vi "1_Waveform_Signal_Regression(Training).vi"() -> ()   [LabVIEW 2020]
uses:
  <vilib>/Ngene/Deep Learning Toolkit/Toolkit/NN_Train/Controls/NN_LR_Policy_Cfg.ctl
  <vilib>/Ngene/Deep Learning Toolkit/Toolkit/NN_Train/Controls/NN_LR_Policy_Type.ctl
  <vilib>/Ngene/Deep Learning Toolkit/Toolkit/NN_Train/Controls/NN_Train_Session_Data.ctl
  <vilib>/Ngene/Deep Learning Toolkit/Toolkit/NN_Train/Controls/NN_Train_Params.ctl
  <vilib>/Ngene/Deep Learning Toolkit/Toolkit/NN_Train/Controls/NN_Train_Optimizer.ctl
  <vilib>/Ngene/Deep Learning Toolkit/Toolkit/NN_Train/Controls/NN_Train_Data_Sampling.ctl
  <vilib>/Ngene/Deep Learning Toolkit/Toolkit/NN_Network/Controls/NN_Device.ctl
  <vilib>/Ngene/Deep Learning Toolkit/Toolkit/NN_Layers/Layers/Input/Controls/NN_Layer_Config(Input1D).ctl
  <vilib>/Ngene/Deep Learning Toolkit/Toolkit/NN_Data/Controls/NN_Data_type.ctl
  <vilib>/Ngene/Deep Learning Toolkit/Toolkit/NN_Layers/Layers/FC/Controls/NN_Layer_Config(FC).ctl
  <vilib>/Ngene/Deep Learning Toolkit/Toolkit/NN_Layers/Layers/BatchNorm/Controls/NN_BN_Params.ctl
  <vilib>/Ngene/Deep Learning Toolkit/Toolkit/NN_Activations/Controls/NN_Activation_Type.ctl
  <vilib>/Ngene/Deep Learning Toolkit/Toolkit/NN_Layers/Controls/NN_Layer_Init_Params.ctl
  <vilib>/Ngene/Deep Learning Toolkit/Toolkit/NN_Layers/Controls/NN_Layer_Weight_Init_Type.ctl
  <vilib>/Ngene/Deep Learning Toolkit/Toolkit/NN_Network/Controls/NN_Save_Before_Destroy_Options.ctl
  <vilib>/Ngene/Deep Learning Toolkit/Toolkit/NN_Layers/Layers/Input/NN_Layer_Create(Input1D).vi
  <vilib>/Ngene/Deep Learning Toolkit/Toolkit/NN_Layers/Layers/FC/NN_Layer_Create(FC).vi
  <vilib>/Ngene/Deep Learning Toolkit/Toolkit/NN_Train/Eval_Loss/NN_Eval_Test_Error_Loss/NN_Eval(In1D_Out1D).vi
  <vilib>/Ngene/Deep Learning Toolkit/Toolkit/NN_Train/Loss_Functions/NN_Set_Loss(MSE).vi
  <vilib>/Ngene/Deep Learning Toolkit/Toolkit/NN_Network/subVIs/NN_Predict/NN_Predict(In1D_Out1D).vi
  <vilib>/Ngene/Deep Learning Toolkit/Toolkit/Deep_Learning_Toolkit_by_Ngene.lvlib
  <vilib>/ptbypt/NI_PtbyPt.lvlib
panel:
  out "Training Loss":sgl=30.107077 format="%#.6g"
  in  "Eval":bool
  out "Loss Graphs":cluster{"mean":dbl, "Test Loss":sgl}(graph)
  in  "NN_Device":T1=enum."GPU"
  out "Test Loss":sgl=0.33381224 format="%#.6g"
  in  "Stop Training":bool
  in  "NN_Train_Params":T2={"Optimizer"=enum."Adam", "Beta_1"=0.9, "Beta_2"=0.999, "Weight Decay(L1)"=1e-07, "Weight Decay(L2)"=1e-07, "Data_Sampling"=enum."Random"}
  out "Session Data":T5={"Epochs"=22.1088, "Tot_Iter"=13818, "LR"=0.0025, "LR_iter"=13819}
  in  "LR Update Policy":T6={"Policy_Type"=enum."Step", "LR0"=0.010000000000000002, "k"=10.0, "WarmUp_Policy"=enum."Ramp", "WarmUp_Iter"=1000, "WarmUp_Ratio"=100.0} {"WarmUp_Ratio" min=1; "WarmUp_Iter" min=1; "LR0" format="%.7f"}
  # "Overview: This example demonstrating the usage of Deep Learning Toolkit for solving  waveform signal regression problem.\nRequirements: Deep Learning Toolkit for LabVIEW\nInstructions:\n1.  Run the VI with current configuration of the training parameters and Learning Rate update policy.\n2. Observe how the training loss is decreasing.\n3. Press the \"Stop Training\" when the loss is not decreasing any more."
  # "Waveform Signal Regression (Frequency Prediction) - Training"
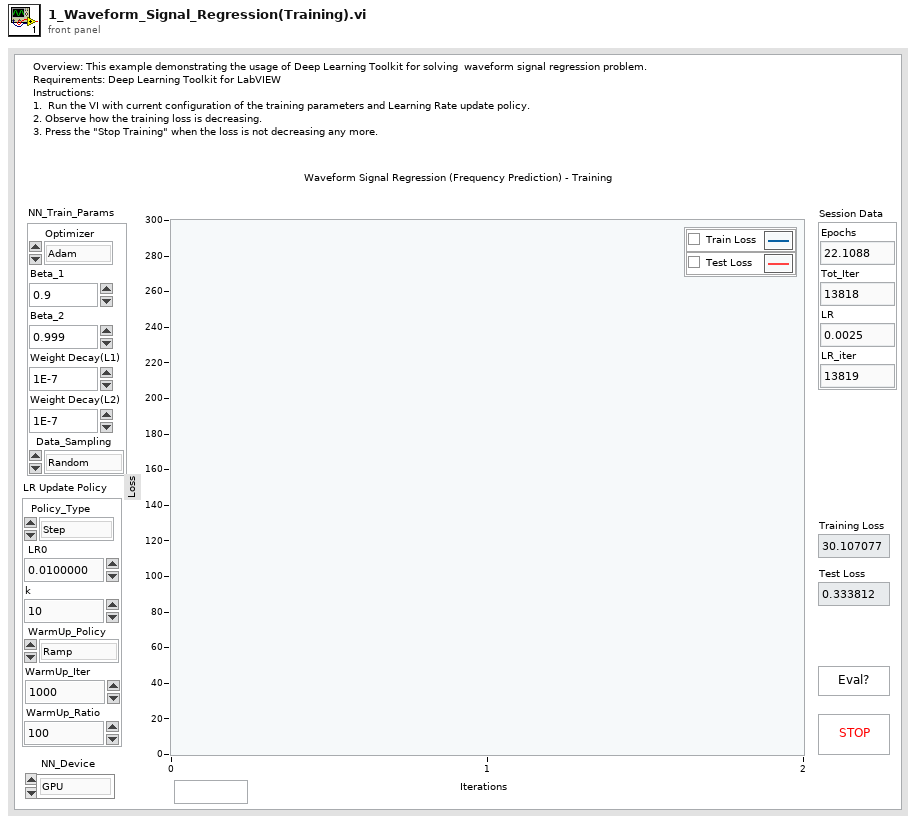
[diagram p1: front panel]
types:
  T1 = typedef "Deep_Learning_Toolkit_by_Ngene.lvlib/NN_Device.ctl" = enum16{"CPU", "GPU"}
  T2 = typedef "Deep_Learning_Toolkit_by_Ngene.lvlib/NN_Train_Params.ctl" = cluster{"Optimizer":T3, "Beta_1":sgl, "Beta_2":sgl, "Weight Decay(L1)":sgl, "Weight Decay(L2)":sgl, "Data_Sampling":T4}
  T3 = typedef "Deep_Learning_Toolkit_by_Ngene.lvlib/NN_Train_Optimizer.ctl" = enum16{"SGD", "Adam", "Adagrad", "Adadelta", "RMSProp", "Nesterov"}
  T4 = typedef "Deep_Learning_Toolkit_by_Ngene.lvlib/NN_Train_Data_Sampling.ctl" = enum16{"Random", "Sequential"}
  T5 = typedef "Deep_Learning_Toolkit_by_Ngene.lvlib/NN_Train_Session_Data.ctl" = cluster{"Epochs":sgl, "Tot_Iter":i32, "LR":sgl, "LR_iter":i32}
  T6 = typedef "Deep_Learning_Toolkit_by_Ngene.lvlib/NN_LR_Policy_Cfg.ctl" = cluster{"Policy_Type":T7, "LR0":dbl, "k":sgl, "WarmUp_Policy":enum16{"Step", "Ramp"}, "WarmUp_Iter":i32, "WarmUp_Ratio":sgl}
  T7 = typedef "Deep_Learning_Toolkit_by_Ngene.lvlib/NN_LR_Policy_Type.ctl" = enum16{"Manual", "Step", "Exp", "1/t"}
  T8 = typedef "Deep_Learning_Toolkit_by_Ngene.lvlib/NN_Save_Before_Destroy_Options.ctl" = cluster{"CFG?":bool, "Weights?":bool, "Render?":bool}
  T9 = typedef "Deep_Learning_Toolkit_by_Ngene.lvlib/NN_Layer_Config(FC).ctl" = cluster{"Name":string, "Size":i32, "BN":bool, "BN_Params":T10, "Activation":T11, "Has Bias?":bool, "Init_Params":T12, "Custom_Params":string}
  T10 = typedef "Deep_Learning_Toolkit_by_Ngene.lvlib/NN_BN_Params.ctl" = cluster{"epsilon":sgl, "momentum":sgl}
  T11 = typedef "Deep_Learning_Toolkit_by_Ngene.lvlib/NN_Activation_Type.ctl" = enum16{"Sigmoid", "ReLU", "LReLU", "ReLU6", "GELU", "tanh", "Swish", "Mish", "None"}
  T12 = typedef "Deep_Learning_Toolkit_by_Ngene.lvlib/NN_Layer_Init_Params.ctl" = cluster{"Init_Type":T13, "Value":sgl}
  T13 = typedef "Deep_Learning_Toolkit_by_Ngene.lvlib/NN_Layer_Weight_Init_Type.ctl" = enum16{"Const", "Uniform", "Gaussian", "Xavier"}
  T14 = typedef "Deep_Learning_Toolkit_by_Ngene.lvlib/NN_Layer_Config(Input1D).ctl" = cluster{"Name":string, "Size":i32, "Data_Type":T15, "Shift":sgl, "Scale":sgl}
  T15 = typedef "Deep_Learning_Toolkit_by_Ngene.lvlib/NN_Data_type.ctl" = enum16{"I8", "U8", "I16", "U16", "U32 ARGB", "SGL"}
  T16 = typedef "Deep_Learning_Toolkit_by_Ngene.lvlib/NN_DataSets_All(In1D_Out1D).ctl" = cluster{"Train":T17, "Validation":T17, "Test":T17}
  T17 = typedef "Deep_Learning_Toolkit_by_Ngene.lvlib/NN_DataSet(In1D_Out1D).ctl" = cluster{"Inputs Ref.":variant, "Outputs Ref.":T18, "Dims_In":i32, "Dataset_Size":i32, "Dims_Out":i32, "Labels":string[], "File Paths":path[], "Custom_Data":variant}
  T18 = typedef "Deep_Learning_Toolkit_by_Ngene.lvlib/NN_Data_ref(2D_SGL).ctl" = refnum<data-value>
  T19 = typedef "Deep_Learning_Toolkit_by_Ngene.lvlib/NN.ctl" = cluster{"Name":string, "No of Layers":i32, "mBatch":i32, "Layers":T20[], "Dimty":T21, "Dims_In":T22, "Dims_Out":T22, "Working_Dir":path, "Train?":bool, "Train_Params":T2, "LR_Update_Policy":T6, "Session Data":T5, "Ground_truth":T23, "NNg_hdls":T24, "NN_Device":T1, "GPU Id":i32, "Labels":string[], "Loss_Type":T25, "Loss_Cfg_Prms":variant, "NNG_WS":T26, "DryRun?":bool}
  T20 = typedef "Deep_Learning_Toolkit_by_Ngene.lvlib/NN_Layer_ref.ctl" = refnum<file>
  T21 = typedef "Deep_Learning_Toolkit_by_Ngene.lvlib/NN_In_Out_Dim-ty.ctl" = enum8{"In1D_Out1D", "In3D_Out1D", "In3D_Out3D", "In3D_OutBBox"}
  T22 = typedef "Deep_Learning_Toolkit_by_Ngene.lvlib/NN_Dims(C,H,W).ctl" = cluster{"C":i32, "H":i32, "W":i32}
  T23 = typedef "Deep_Learning_Toolkit_by_Ngene.lvlib/NN_Ground_truth.ctl" = cluster{"Y":variant}
  T24 = typedef "Deep_Learning_Toolkit_by_Ngene.lvlib/nng_cuda_handles.ctl" = cluster{"cudnn":u64, "cublas":u64, "stream":u64, "curand":u64}
  T25 = typedef "Deep_Learning_Toolkit_by_Ngene.lvlib/NN_Loss_Type.ctl" = enum16{"None", "MSE", "CrossEntropy", "YOLO_v2", "YOLO_v4"}
  T26 = typedef "Deep_Learning_Toolkit_by_Ngene.lvlib/NNG_WS.ctl" = cluster{"NNG_WS_Mem":T27, "Max_WS_Size":i64}
  T27 = typedef "Deep_Learning_Toolkit_by_Ngene.lvlib/NNg_WS_Mem_DVR.ctl" = refnum<data-value>
  T28 = typedef "Deep_Learning_Toolkit_by_Ngene.lvlib/NN_Eval_Params.ctl" = cluster{"Loss":sgl, "Error":sgl}
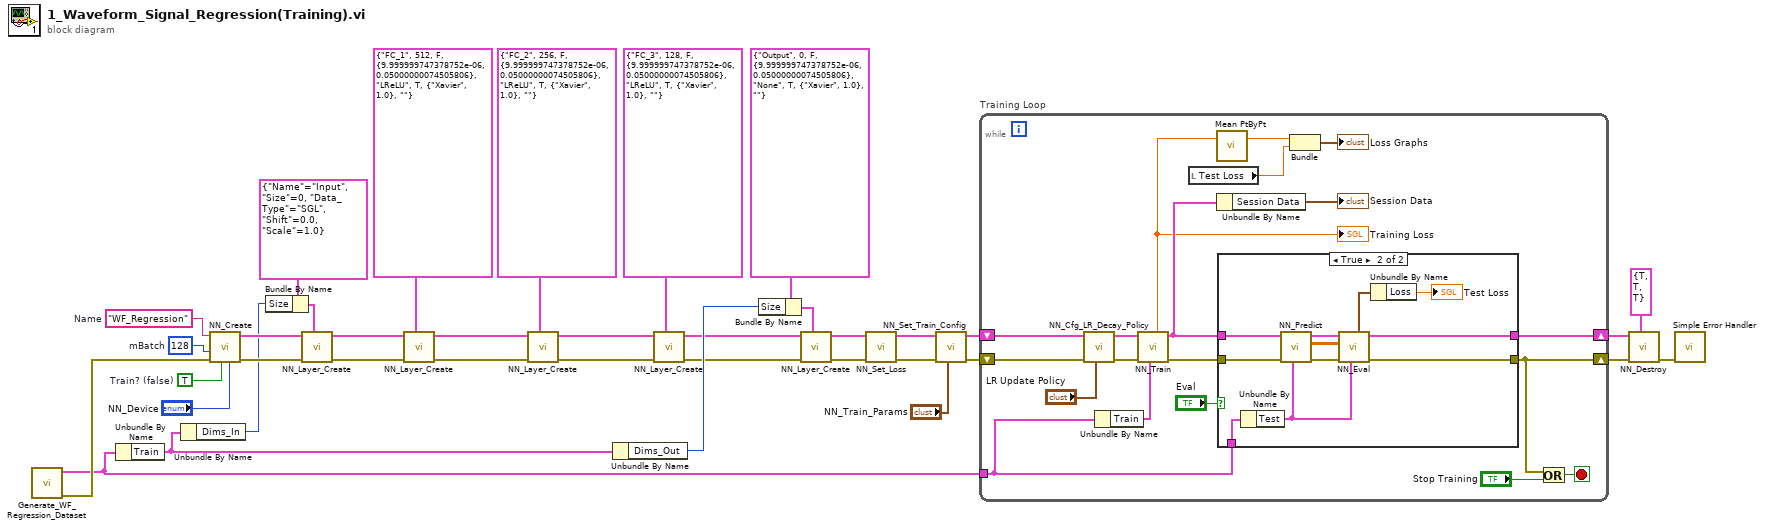
[diagram p0: block diagram]
diagram:
  w18 = "WF_Regression"  # Name
  w19 = 128  # mBatch
  w20 = TRUE  # Train? (false)
  n1 = call "Generate_WF_Regression_Dataset.vi"() -> ("error out"=w29:errorcluster, "DataSets_All(In1D_Out1D)"=w3:T16)  [unwired: 10 in]
  n2 = Unbundle By Name(w3) -> ("Train"=w1:T17)
  n3 = Unbundle By Name(w1) -> ("Dims_In"=w27:i32)
  n4 = call <vilib>:"NN_Create.vi"("NN_Device"="NN_Device", "Train? (false)"=w20, "error in (no error)"=w29, "mBatch (1)"=w19, "Name"=w18) -> ("error out"=w36:errorcluster, "NN out"=w37:T19)  [unwired: 5 in]
  n5 = Bundle By Name(cluster=T14 {"Name"="Input", "Size"=0, "Data_Type"=enum."SGL", "Shift"=0.0, "Scale"=1.0} ("Input1D_Cfg"), "Size"=w27) -> (w28:T14)
  n6 = call-poly <vilib>:"NN_Layer_Create.vi"("Input1D_Cfg"=w28, "error in (no error)"=w36, "NN in"=w37) -> ("error out"=w23:errorcluster, "NN out"=w24:T19)  [unwired: 6 in, 1 out]
  n7 = call-poly <vilib>:"NN_Layer_Create.vi"("FC_Cfg"=T9 {"Name"="FC_1", "Size"=512, "BN"=FALSE, "BN_Params"={"epsilon"=1e-05, "momentum"=0.05}, "Activation"=enum."LReLU", "Has Bias?"=TRUE, "Init_Params"={"Init_Type"=enum."Xavier", "Value"=1.0}, "Custom_Params"=""} ("FC_Cfg_1"), "error in (no error)"=w23, "NN in"=w24) -> ("error out"=w12:errorcluster, "NN out"=w13:T19)  [unwired: 6 in, 1 out]
  n8 = call-poly <vilib>:"NN_Layer_Create.vi"("FC_Cfg"=T9 {"Name"="FC_2", "Size"=256, "BN"=FALSE, "BN_Params"={"epsilon"=1e-05, "momentum"=0.05}, "Activation"=enum."LReLU", "Has Bias?"=TRUE, "Init_Params"={"Init_Type"=enum."Xavier", "Value"=1.0}, "Custom_Params"=""} ("FC_Cfg_1"), "error in (no error)"=w12, "NN in"=w13) -> ("error out"=w8:errorcluster, "NN out"=w9:T19)  [unwired: 6 in, 1 out]
  n9 = Unbundle By Name(w1) -> ("Dims_Out"=w25:i32)
  n10 = call-poly <vilib>:"NN_Layer_Create.vi"("FC_Cfg"=T9 {"Name"="FC_3", "Size"=128, "BN"=FALSE, "BN_Params"={"epsilon"=1e-05, "momentum"=0.05}, "Activation"=enum."LReLU", "Has Bias?"=TRUE, "Init_Params"={"Init_Type"=enum."Xavier", "Value"=1.0}, "Custom_Params"=""} ("FC_Cfg_1"), "error in (no error)"=w8, "NN in"=w9) -> ("error out"=w6:errorcluster, "NN out"=w7:T19)  [unwired: 6 in, 1 out]
  n11 = Bundle By Name(cluster=T9 {"Name"="Output", "Size"=0, "BN"=FALSE, "BN_Params"={"epsilon"=1e-05, "momentum"=0.05}, "Activation"=enum."None", "Has Bias?"=TRUE, "Init_Params"={"Init_Type"=enum."Xavier", "Value"=1.0}, "Custom_Params"=""} ("FC_Cfg_1"), "Size"=w25) -> (w26:T9)
  n12 = call-poly <vilib>:"NN_Layer_Create.vi"("FC_Cfg"=w26, "error in (no error)"=w6, "NN in"=w7) -> ("error out"=w32:errorcluster, "NN out"=w33:T19)  [unwired: 6 in, 1 out]
  n13 = call-poly <vilib>:"NN_Set_Loss.vi"("error in (no error)"=w32, "NN in"=w33) -> ("error out"=w15:errorcluster, "NN out"=w16:T19)  [unwired: 8 in]
  n14 = call <vilib>:"NN_Set_Train_Config.vi"("NN_Train_Params"="NN_Train_Params", "error in (no error)"=w15, "NN in"=w16) -> ("error out"=w21:errorcluster, "NN out"=w22:T19)  [unwired: 7 in]
  n15 = while "Training Loop" {
    shift-right: [w41] -> w4
    shift-left: w21 -> [w51]
    shift-right: [w47] -> w5
    shift-left: w22 -> [w54]
    tunnel: w3 -> [w39]
    stop <- w42 stop-if-true
    n16 = call <vilib>:"NN_Cfg_LR_Decay_Policy.vi"("LR_Decay_Params"="LR Update Policy", "error in (no error)"=w51, "NN in"=w54) -> ("error out"=w52:errorcluster, "NN out"=w53:T19)  [unwired: 7 in]
    n17 = Unbundle By Name(w39) -> ("Train"=w38:T17)
    n18 = call <vilib>:"NN_Train.vi"("Train Dataset"=w38, "error in (no error)"=w52, "NN in"=w53) -> ("error out"=w48:errorcluster, "NN out"=w49:T19, "Loss"=w43:sgl)  [unwired: 3 in, 3 out]
    "Training Loss" <- w43
    n19 = local read "Test Loss"() -> (w45:sgl)
    n20 = call <vilib>:"Mean PtByPt.vi"("x"=w43) -> ("mean"=w40:dbl)  [unwired: 3 in, 1 out]
    n21 = Unbundle By Name(w49) -> ("Session Data"=→"Session Data":T5)
    n22 = case shown="True" "Eval" {
      tunnel: w49 -> [w58 w68]
      tunnel: w48 -> [w57 w67]
      tunnel: [w58 w66] -> w47
      tunnel: [w57 w63] -> w41
      tunnel: w39 -> [_ w62]
      frame False {
      }
      frame True {
        n23 = Unbundle By Name(w62) -> ("Test"=w61:T17)
        n24 = call-poly <vilib>:"NN_Predict.vi"("Dataset"=w61, "error in (no error)"=w67, "NN in"=w68) -> ("error out"=w69:errorcluster, "Predictions"=w64:sgl[][], "NN out"=w65:T19)  [unwired: 6 in]
        n25 = call-poly <vilib>:"NN_Eval.vi"("Dataset"=w61, "error in (no error)"=w69, "Predictions"=w64, "NN in"=w65) -> ("error out"=w63:errorcluster, "NN out"=w66:T19, "NN_Eval_Params"=w60:T28)  [unwired: 4 in, 1 out]
        n26 = Unbundle By Name(w60) -> ("Loss"=→"Test Loss":sgl)
      }
    }
    n27 = Bundle("mean"=w40, "Test Loss"=w45) -> (→"Loss Graphs":cluster{"mean":dbl, "Test Loss":sgl})  [unwired: 1 in]
    n28 = Or(x=w41, y="Stop Training") -> (x .or. y?=w42:bool)
  }
  n29 = call <vilib>:"NN_Destroy.vi"("Save (T, T, T)"=T8 {"CFG?"=TRUE, "Weights?"=TRUE, "Render?"=TRUE}, "error in (no error)"=w4, "NN in"=w5) -> ("error out"=w31:errorcluster)  [unwired: 7 in, 1 out]
  n30 = call <vilib>:"Simple Error Handler.vi"("error in (no error)"=w31) -> ()  [unwired: 4 in, 5 out]
